vi "Set TP.vi"(8 "error in (no error)":errorcluster, 10 "Main":refnum<vi>) -> (0 "error out":errorcluster)   [LabVIEW 2025, in "Flow Grind.lvlib" / "Leakage.lvclass"]
uses:
  Leakage.lvclass
  Leakage.lvclass/Leakage.ctl
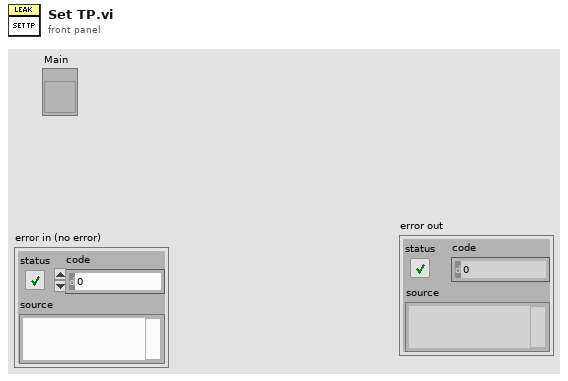
[diagram p1: front panel]
types:
  T1 = cluster{"Name":string, "Color":u32, "Style":u8, "Point Style":u8, "Name Visible":bool, "Allow Drag":bool, "Annotation Mode":u32, "Plot":i32, "Index":i32, "Position":cluster{"X":dbl, "Y":dbl}, "X Scale":u32, "Y Scale":u32, "Show Arrow":bool, "Lock Name":bool, "Plot Area":i32, "Label Offset":cluster{"X":dbl, "Y":dbl}}
  T2 = typedef "LVAnnotationListTypeDef.ctl" = cluster{"Name":string, "Color":u32, "Style":u8, "Point Style":u8, "Name Visible":bool, "Allow Drag":bool, "Annotation Mode":u32, "Plot":i32, "Index":i32, "Position":cluster{"X":dbl, "Y":dbl}, "X Scale":u32, "Y Scale":u32, "Show Arrow":bool, "Lock Name":bool, "Plot Area":i32, "Label Offset":cluster{"X":dbl, "Y":dbl}}[]
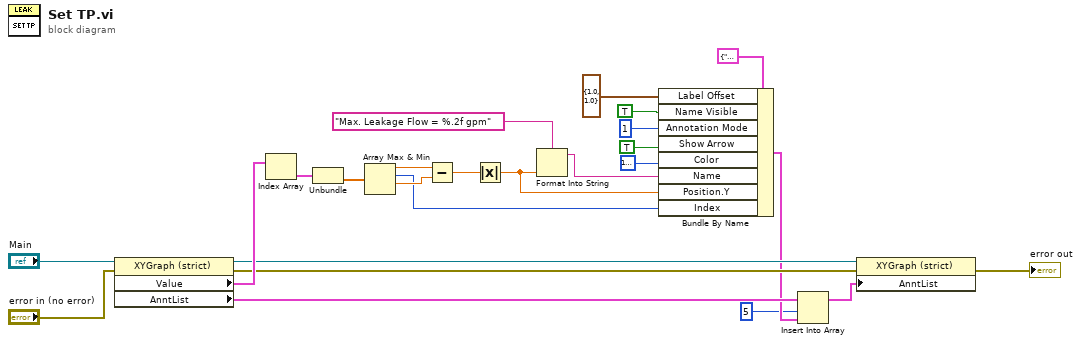
[diagram p0: block diagram]
diagram:
  n1 = property class="XYGraph (strict)"(reference="Main", error in="error in (no error)") -> (reference out=w12:refnum<vi>, error out=w8:errorcluster, "Value"=w23:cluster{dbl[], dbl[]}[], "AnntList"=w5:T2)
  n2 = Index Array(array=w23) -> (element=w22:cluster{dbl[], dbl[]})  [unwired: 1 in]
  n3 = Unbundle(w22) -> (w21:dbl[])  [unwired: 1 out]
  n4 = Array Max & Min(array=w21) -> (max value=w20:dbl, max index (indices)=w10:i32, min value=w19:dbl)  [unwired: 1 out]
  n5 = Subtract(x=w20, y=w19) -> (x-y=w24:dbl)
  n6 = Absolute Value(x=w24) -> (abs(x)=w9:dbl)
  n7 = Format Into String(format string="Max. Leakage Flow = %.2f gpm", w9) -> (resulting string=w11:string)  [unwired: 2 in, 1 out]
  n8 = Bundle By Name(cluster=T1 {"Name"="", "Color"=0, "Style"=0, "Point Style"=0, "Name Visible"=FALSE, "Allow Drag"=FALSE, "Annotation Mode"=0, "Plot"=0, "Index"=0, "Position"={"X"=0.0, "Y"=0.0}, "X Scale"=0, "Y Scale"=0, "Show Arrow"=FALSE, "Lock Name"=FALSE, "Plot Area"=0, "Label Offset"={"X"=0.0, "Y"=0.0}}, "Label Offset"=cluster{"X":dbl, "Y":dbl} {"X"=1.0, "Y"=1.0}, "Name Visible"=TRUE, "Annotation Mode"=u32 1, "Show Arrow"=TRUE, "Color"=u32 16777224, "Name"=w11, "Position.Y"=w9, "Index"=w10) -> (w4:T1)
  n9 = Insert Into Array(array=w5, index=5, new element=w4) -> (w3:T2)
  n10 = property class="XYGraph (strict)"(reference=w12, error in=w8, "AnntList"=w3) -> (error out=→"error out":errorcluster)  [unwired: 1 out]
